vi "CloseModuleManager.vi"(8 "error in (no error)":errorcluster, 11 "Sensor Engine Datas in":T1[](array[typedef])) -> (0 "error out":errorcluster)   [LabVIEW 2023, in "MM.lvlib"]
uses:
  MM.lvlib
  Sensor Engine Data.ctl
  DataContainer/DataContainer.lvclass
  Shared/Protocol.ctl
  Shared/Vires VTD Shared.lvlib
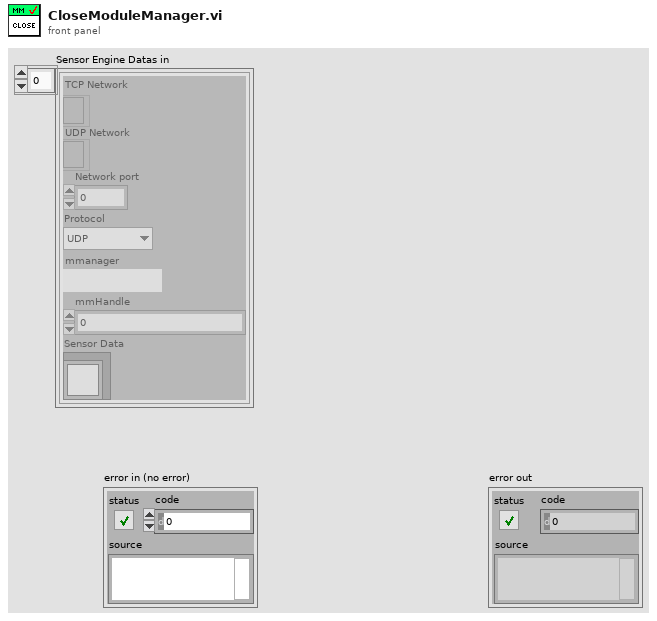
[diagram p1: front panel]
types:
  T1 = typedef "MM.lvlib/Sensor Engine Data.ctl" = cluster{"TCP Network":refnum<k5>, "UDP Network":refnum<k16>, "Network port":i32, "Protocol":T2, "mmanager":path, "mmHandle":u64, "Sensor Data":refnum<class "DataContainer.lvclass">}
  T2 = typedef "Vires VTD Shared.lvlib/Protocol.ctl" = enum16{"UDP", "TCP"}
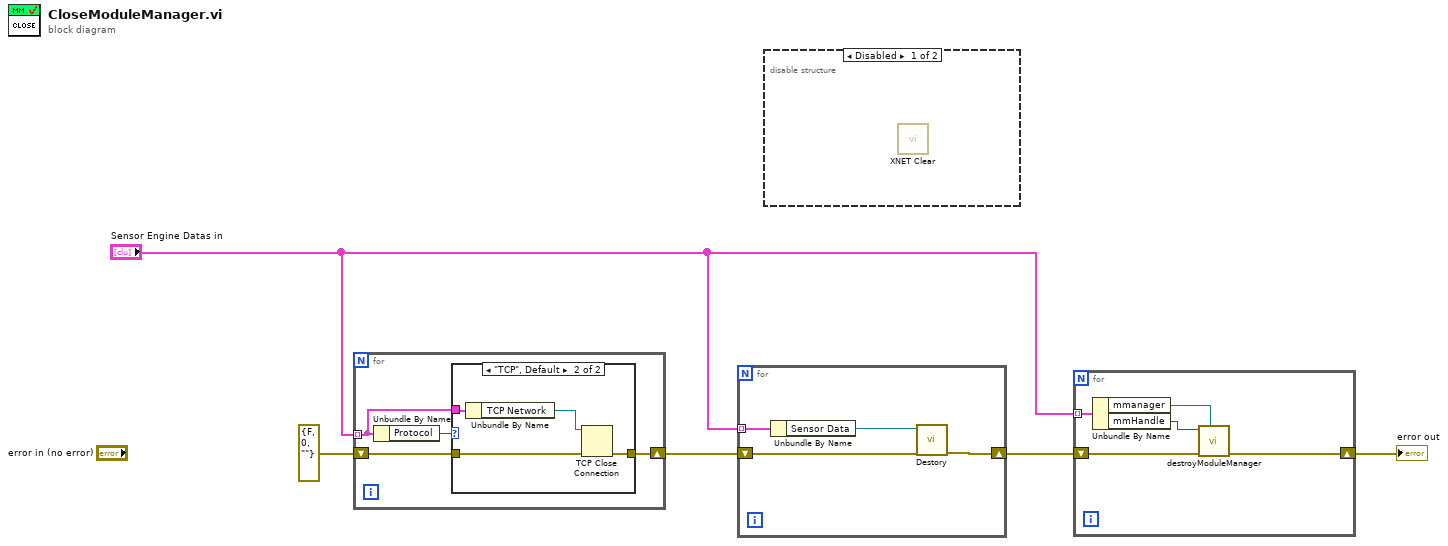
[diagram p0: block diagram]
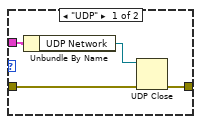
[diagram p3: hidden frame]
diagram:
  n1 = for {
    shift-right: [w8] -> w5
    shift-left: errorcluster {"status"=FALSE, "code"=0, "source"=""} ("error out") -> [w9]
    tunnel: "Sensor Engine Datas in" -> [w6] mode=indexing
    n2 = Unbundle By Name(w6) -> ("Protocol"=w7:T2)
    n3 = case shown="\"TCP\", Default" w7 {
      tunnel: w9 -> [w12 w17]
      tunnel: [w11 w16] -> w8
      tunnel: w6 -> [w13 w15]
      frame "UDP" {
        n4 = Unbundle By Name(w13) -> ("UDP Network"=w10:refnum<k16>)
        n5 = UDP Close(connection ID=w10, 8:w12) -> (error out=w11:errorcluster)  [unwired: 1 out]
      }
      frame "TCP", Default {
        n6 = Unbundle By Name(w15) -> ("TCP Network"=w14:refnum<k5>)
        n7 = TCP Close Connection(connection ID=w14, error in (no error)=w17) -> (error out=w16:errorcluster)  [unwired: 1 in, 1 out]
      }
    }
  }
  n8 = for {
    shift-right: [w20] -> w2
    shift-left: w5 -> [w21]
    tunnel: "Sensor Engine Datas in" -> [w19] mode=indexing
    n9 = Unbundle By Name(w19) -> ("Sensor Data"=w18:refnum<class "DataContainer.lvclass">)
    n10 = call-dynamic "Destory.vi"("error in (no error)"=w21, "DataContainer in"=w18) -> ("error out"=w20:errorcluster)  [unwired: 8 in, 1 out]
  }
  n11 = disable-structure shown="Disabled" {
    frame Disabled {
      n12 = call <vilib>:"XNET Clear.vi"() -> ()  [unwired: 15 in, 1 out]
    }
    frame Enabled {
    }
  }
  n13 = for {
    tunnel: "Sensor Engine Datas in" -> [w26] mode=indexing
    shift-right: [w22] -> w1
    shift-left: w2 -> [w23]
    n14 = Unbundle By Name(w26) -> ("mmanager"=w25:path, "mmHandle"=w24:u64)
    n15 = call "destroyModuleManager.vi"("path in"=w25, "error in (no error)"=w23, "mmHandle"=w24) -> ("error out"=w22:errorcluster)  [unwired: 8 in]
  }
  "error out" <- w1
